vi "Enable HTTPS.vi"(7 "Private Key Password (None)":string, 8 "error in (no error)":errorcluster, 10 "HTTPS Options":T1={"HTTPS Enabled"=FALSE, "Private Key"=path "", "Private Key Format"=enum."PKCS#8 (PEM)", "Public Cert"=path "", "Public Cert Format"=enum."X.509 (PEM)", "Always Secure?"=TRUE, "HTTPS Port (443)"=433}, 11 "Server in":refnum<class "Server.lvclass">) -> (0 "error out":errorcluster, 3 "Server out":refnum<class "Server.lvclass">)   [LabVIEW 2020, in "HTTP Server.lvlib" / "Server.lvclass"]
uses:
  Server.lvclass
  Server.lvclass/Server.ctl
  lv-uri/URI/URI/URI.lvclass
  HTTPS Options.ctl
  HTTP Server.lvlib
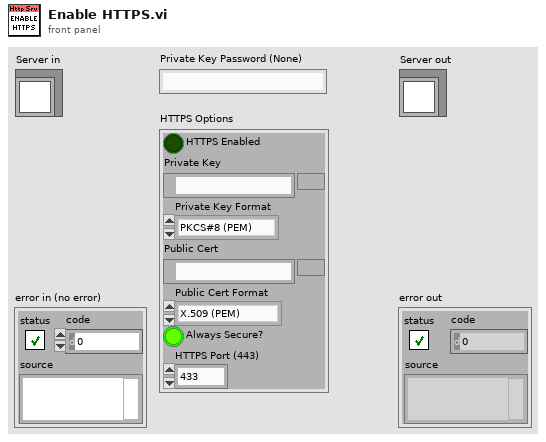
[diagram p1: front panel]
types:
  T1 = typedef "HTTP Server.lvlib/HTTPS Options.ctl" = cluster{"HTTPS Enabled":bool, "Private Key":path, "Private Key Format":enum32{"PKCS#8 (PEM)", "PKCS#8 (DER)"}, "Public Cert":path, "Public Cert Format":enum32{"X.509 (PEM)"}, "Always Secure?":bool, "HTTPS Port (443)":u16}
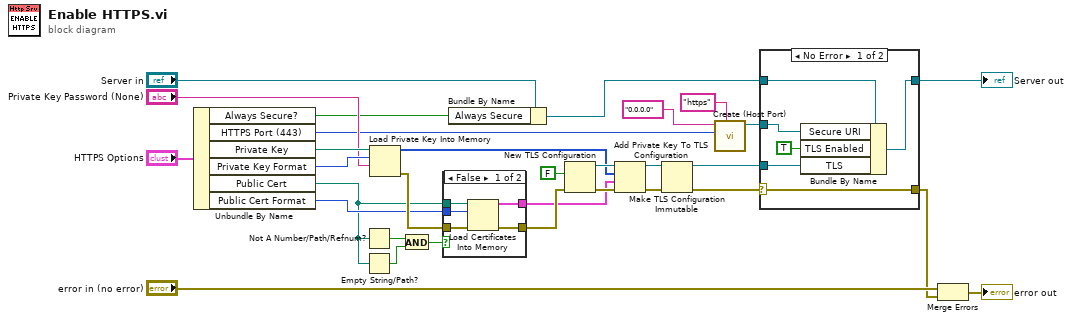
[diagram p0: block diagram]
diagram:
  n1 = Unbundle By Name("HTTPS Options") -> ("Always Secure?"=w9:bool, "HTTPS Port (443)"=w4:u16, "Private Key"=w27:path, "Private Key Format"=w26:enum32{"PKCS#8 (PEM)", "PKCS#8 (DER)"}, "Public Cert"=w8:path, "Public Cert Format"=w21:enum32{"X.509 (PEM)"})
  n2 = Not A Number/Path/Refnum?(number/path/refnum=w8) -> (NaN/Path/Refnum?=w7:bool)
  n3 = Empty String/Path?(string/path=w8) -> (empty?=w6:bool)
  n4 = Load Private Key Into Memory(9:"Private Key Password (None)", 10:w26, 11:w27) -> (0:w31:errorcluster, 3:w22:u8[])  [unwired: 1 in]
  n5 = And(x=w7, y=w6) -> (x .and. y?=w5:bool)
  n6 = case shown="False" w5 {
    tunnel: w31 -> [w36 w37]
    tunnel: [w35 w37] -> w30
    tunnel: w21 -> [w34 _]
    tunnel: [w33 _] -> w20
    tunnel: w8 -> [w32 _]
    frame False {
      n7 = Load Certificates Into Memory(8:w36, 10:w34, 11:w32) -> (0:w35:errorcluster, 3:w33:cluster{"certificate":u8[]}[])
    }
    frame True {
    }
  }
  n8 = Bundle By Name(cluster="Server in", "Always Secure"=w9) -> (w10:refnum<class "Server.lvclass">)
  n9 = New TLS Configuration(8:w30, 10:FALSE ("load OS trusted CAs?")) -> (0:w23:errorcluster, 3:w24:refnum<k36>)
  n10 = Add Private Key To TLS Configuration(8:w23, 9:w20, 10:w22, 11:w24) -> (0:w18:errorcluster, 3:w19:refnum<k36>)
  n11 = Make TLS Configuration Immutable(8:w18, 11:w19) -> (0:w17:errorcluster, 3:w15:refnum<k36>)
  n12 = call "Create (Host Port).vi"("Scheme (None)"="https", "Port"=w4, "Host"="0.0.0.0") -> ("URI out"=w3:refnum<class "URI.lvclass">)  [unwired: 8 in]
  n13 = case shown="No Error" w17 {
    selector: w17 -> [w42 w45]
    tunnel: w10 -> [w40 w44]
    tunnel: w15 -> [w43 _]
    tunnel: [w41 w44] -> w14
    tunnel: [w42 w45] -> w11
    tunnel: w3 -> [w38 _]
    frame No Error {
      n14 = Bundle By Name(cluster=w40, "Secure URI"=w38, "TLS Enabled"=TRUE, "TLS"=w43) -> (w41:refnum<class "Server.lvclass">)
    }
    frame Error {
    }
  }
  "Server out" <- w14
  n15 = Merge Errors("error in (no error)", w11) -> (→"error out":errorcluster)
